vi "variant to i32.vi"(1 "Variant":variant) -> (0 "I32":i32)   [LabVIEW 2025]
doc: "convert variant data to a LabVIEW 4-Byte signed Integer (I32)\n<B>Input:</B>\nVariant (skalar)\n<B>Output:</B>\n4-Byte signed Integer (I32)"
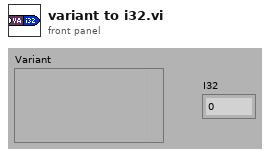
[diagram p1: front panel]
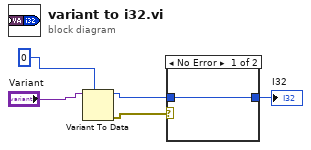
[diagram p0: block diagram]
diagram:
  n1 = Variant To Data(type=0 ("MIN U/36V"), Variant="Variant") -> (data=w3:i32, error out=w4:errorcluster)  [unwired: 1 in]
  n2 = case shown="No Error" w4 {
    tunnel: w3 -> [w6 _]
    tunnel: [w6 _] -> w5
    frame No Error {
    }
    frame Error {
    }
  }
  "I32" <- w5
